vi "Read Test Report.vi"(11 "Test Runner in":refnum<class "Test Runner.lvclass">) -> (1 "defined":bool, 2 "Test Report":refnum<class "Test Report.lvclass">, 3 "Test Runner out":refnum<class "Test Runner.lvclass">)   [LabVIEW 2020, in "Caraya.lvlib" / "Test Runner.lvclass"]
uses:
  Test Runner.lvclass
  Test Report/Test Report.lvclass
  Test Runner.lvclass/Test Runner.ctl
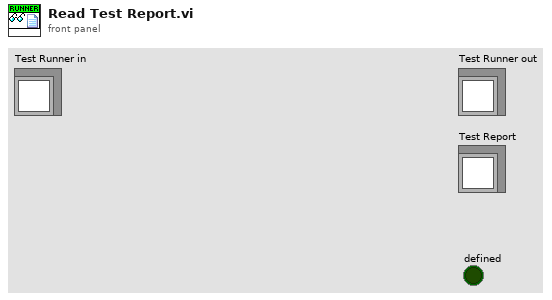
[diagram p1: front panel]
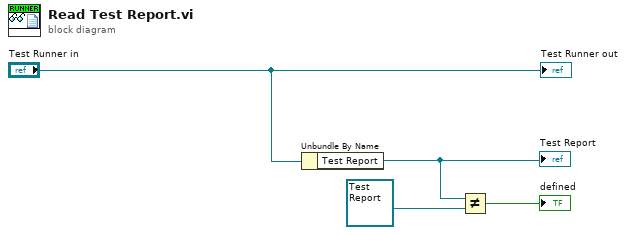
[diagram p0: block diagram]
diagram:
  n1 = Unbundle By Name("Test Runner in") -> ("Test Report"=w3:refnum<class "Test Report.lvclass">)
  "Test Report" <- w3
  n2 = Not Equal?(x=w3, y=refnum<class "Test Report.lvclass"> refnum ("Test Report")) -> (x != y?=→"defined":bool)
  "Test Runner out" <- "Test Runner in"
